vi "~ct - type code convertion (DBL to CDB).vi"(4 "type":T1=enum."CDB Number") -> (1 "type out":T1=enum."DBL Number")   [LabVIEW 2021]
doc: "::: CalcExpress Toolkit :::\nCopyright (c) 2000-2026 Konstantin Shifershteyn. All rights reserved."
uses:
  cetypes.llb/CalcExpress Data Type.ctl
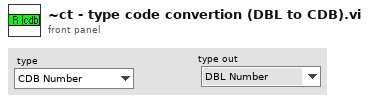
[diagram p1: front panel]
types:
  T1 = typedef "CalcExpress Data Type.ctl" = enum32{"String", "DBL Number", "identifier", "1D Array of DBL", "2D Array of DBL", "CDB Number", "1D Array of CDB", "2D Array of CDB", "1D Array of String", "2D Array of String", "Unknown data type"}
  T2 = enum32{"String", "DBL Number", "identifier", "1D Array of DBL", "2D Array of DBL", "CDB Number", "1D Array of CDB", "2D Array of CDB", "1D Array of String", "2D Array of String", "Unknown data type"}[]
  T3 = enum32{"String", "DBL Number", "identifier", "1D Array of DBL", "2D Array of DBL", "CDB Number", "1D Array of CDB", "2D Array of CDB", "1D Array of String", "2D Array of String", "Unknown data type"}
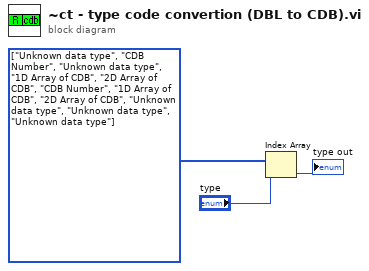
[diagram p0: block diagram]
diagram:
  w3 = T2 [enum."Unknown data type", enum."CDB Number", enum."Unknown data type", enum."1D Array of CDB", enum."2D Array of CDB", enum."CDB Number", enum."1D Array of CDB", enum."2D Array of CDB", enum."Unknown data type", enum."Unknown data type", enum."Unknown data type"] items=["String", "DBL Number", "identifier", "1D Array of DBL", "2D Array of DBL", "CDB Number", "1D Array of CDB", "2D Array of CDB", "1D Array of String", "2D Array of String", "Unknown data type"]
  n1 = Index Array(array=w3, index="type") -> (element=→"type out":T3)
